vi "Test Get Menu Action.vi"() -> ()   [LabVIEW 2026]
doc: "Caraya unit test for Get Menu Action.vi.\n\nOne static subVI call per case. All cases share ONE fixture menu - the application's main menu as Get Main Menu.vi returns it since feature #47 (Fast Cash $100 top left, Fast Cash $50 bottom right). The Menu constant is an instance of the typedef ATM Menu.ctl and every expected constant an instance of ATM States.ctl, so they follow the typedefs when the states enum grows. Do not replace them with unlinked copies: Caraya compares the enum's item list too, and a stale copy fails every case although the numbers are equal.\n\nCase 1: top right button (Right, index 0) selects Deposit Prompt.\nCase 2: middle left button (Left, index 1) selects Balance Inquiry.\nCase 3: no button (index -1) returns None.\nCase 4: top left button (Left, index 0) selects Fast Cash $100.\nCase 5: bottom right button (Right, index 2) still selects Fast Cash, the $50 state.\n\nEvery assertion takes its error in from Define Test rather than from the assertion before it, so a failing case cannot stop a later one. The error cluster carries the FIRST failure only. Read the JUnit report for all of them."
uses:
  Controls/ATM Menu.ctl
  Controls/ATM Menu Side.ctl
  Controls/ATM Menu Item.ctl
  Controls/ATM States.ctl
  <vilib>/addons/_JKI Toolkits/Caraya/classes/Test/Test.lvclass
  <vilib>/addons/_JKI Toolkits/Caraya/classes/Assert/Assert.lvclass
panel:
  out "error out":errorcluster
  in  "error in":errorcluster
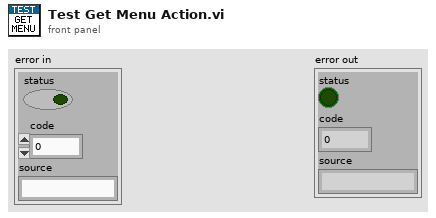
[diagram p1: front panel]
types:
  T1 = typedef "ATM States.ctl" = enum16{"Initialize", "Wait for Event", "Card Inserted", "Process Input", "Verify Account", "Show Main Menu", "Deposit Prompt", "Withdraw Prompt", "Deposit", "Withdraw", "Fast Cash", "Balance Inquiry", "None", "Terminate Session", "Exit", "Fast Cash $100"}
  T2 = typedef "ATM Menu.ctl" = cluster{"Left":T3, "Right":T3}
  T3 = typedef "ATM Menu Side.ctl" = cluster{"Item 1":T4, "Item 2":T4, "Item 3":T4}
  T4 = typedef "ATM Menu Item.ctl" = cluster{"Label":string, "Action":T1}
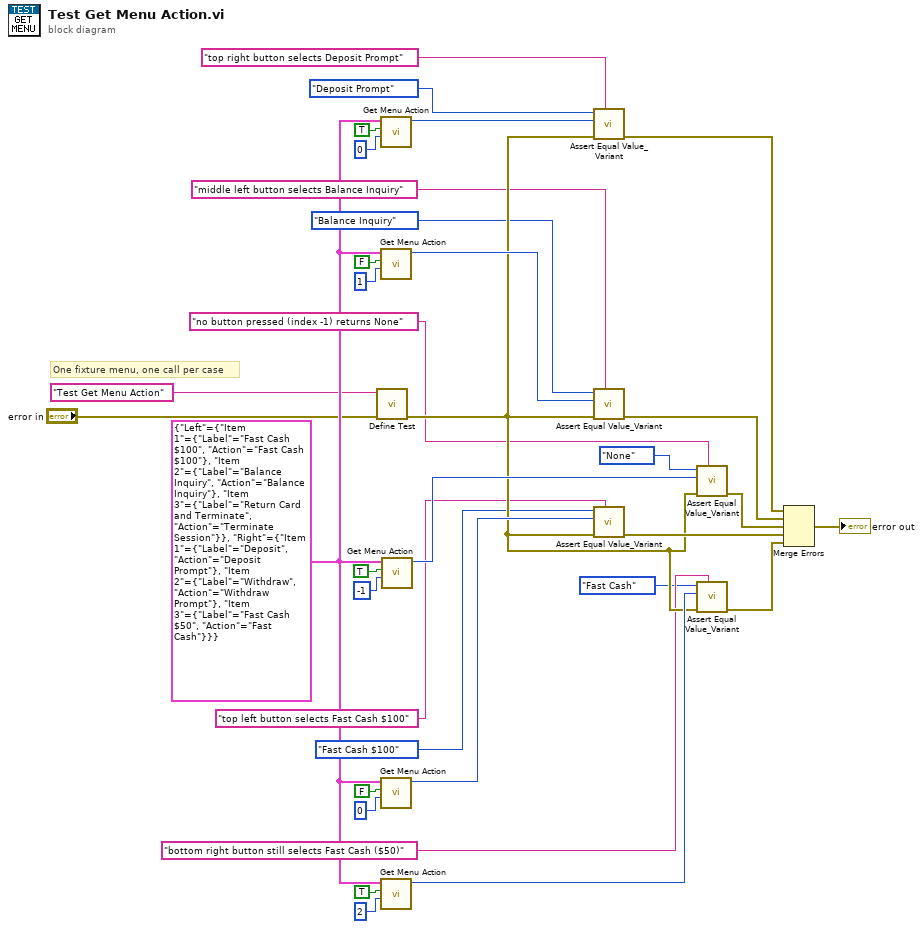
[diagram p0: block diagram]
diagram:
  w4 = T2 {"Left"={"Item 1"={"Label"="Fast Cash $100", "Action"=enum."Fast Cash $100"}, "Item 2"={"Label"="Balance Inquiry", "Action"=enum."Balance Inquiry"}, "Item 3"={"Label"="Return Card and Terminate", "Action"=enum."Terminate Session"}}, "Right"={"Item 1"={"Label"="Deposit", "Action"=enum."Deposit Prompt"}, "Item 2"={"Label"="Withdraw", "Action"=enum."Withdraw Prompt"}, "Item 3"={"Label"="Fast Cash $50", "Action"=enum."Fast Cash"}}} ("Menu")
  # "One fixture menu, one call per case"
  n1 = call <vilib>:"Define Test.vi"("error in (no error)"="error in", "Label (VI Title)"="Test Get Menu Action") -> ("error out"=w25:errorcluster)  [unwired: 8 in, 1 out]
  n2 = call "Get Menu Action.vi"("Button Index"=0 ("Button Index 1"), "Right Side?"=TRUE ("Right Side? 1"), "Menu"=w4) -> ("Action"=w26:T1)  [unwired: 7 in, 1 out]
  n3 = call "Get Menu Action.vi"("Button Index"=1 ("Button Index 2"), "Right Side?"=FALSE ("Right Side? 2"), "Menu"=w4) -> ("Action"=w27:T1)  [unwired: 7 in, 1 out]
  n4 = call "Get Menu Action.vi"("Button Index"=0 ("Button Index 4"), "Right Side?"=FALSE ("Right Side? 4"), "Menu"=w4) -> ("Action"=w29:T1)  [unwired: 7 in, 1 out]
  n5 = call "Get Menu Action.vi"("Button Index"=2 ("Button Index 5"), "Right Side?"=TRUE ("Right Side? 5"), "Menu"=w4) -> ("Action"=w30:T1)  [unwired: 7 in, 1 out]
  n6 = call "Get Menu Action.vi"("Button Index"=-1 ("Button Index 3"), "Right Side?"=TRUE ("Right Side? 3"), "Menu"=w4) -> ("Action"=w28:T1)  [unwired: 7 in, 1 out]
  n7 = call <vilib>:"Assert Equal Value_Variant.vi"("Label"="top right button selects Deposit Prompt" ("Label 1"), "error in (no error)"=w25, "Actual"=w26, "Expected"=ATM_States."Deposit Prompt" ("expected 1")) -> ("error out"=w31:errorcluster)  [unwired: 6 in, 1 out]
  n8 = call <vilib>:"Assert Equal Value_Variant.vi"("Label"="middle left button selects Balance Inquiry" ("Label 2"), "error in (no error)"=w25, "Actual"=w27, "Expected"=ATM_States."Balance Inquiry" ("expected 2")) -> ("error out"=w32:errorcluster)  [unwired: 6 in, 1 out]
  n9 = call <vilib>:"Assert Equal Value_Variant.vi"("Label"="top left button selects Fast Cash $100" ("Label 4"), "error in (no error)"=w25, "Actual"=w29, "Expected"=ATM_States."Fast Cash $100" ("expected 4")) -> ("error out"=w34:errorcluster)  [unwired: 6 in, 1 out]
  n10 = call <vilib>:"Assert Equal Value_Variant.vi"("Label"="no button pressed (index -1) returns None" ("Label 3"), "error in (no error)"=w25, "Actual"=w28, "Expected"=ATM_States."None" ("expected 3")) -> ("error out"=w33:errorcluster)  [unwired: 6 in, 1 out]
  n11 = call <vilib>:"Assert Equal Value_Variant.vi"("Label"="bottom right button still selects Fast Cash ($50)" ("Label 5"), "error in (no error)"=w25, "Actual"=w30, "Expected"=ATM_States."Fast Cash" ("expected 5")) -> ("error out"=w35:errorcluster)  [unwired: 6 in, 1 out]
  n12 = Merge Errors(w31, w32, w33, w34, w35) -> (→"error out":errorcluster)
